vi "IMU Get Yaw Flat.vi"(7 "Alignment Angle":dbl=nan, 8 "error in (no error)":errorcluster, 10 "Units":enum16{"Radians", "Degrees"}(ring)) -> (0 "error out":errorcluster, 2 "timestamp out":i64, 3 "yaw":dbl(graph))   [LabVIEW 2023, in "MrcLib.lvlib"]
doc: "Return the yaw of the built-in sensor in the indicated units assuming it is mounted flat/horizontal relative to the ground (very common). To align with a existing coordinate system, make a call passing in the expected alignment angle."
uses:
  <vilib>/MRC/MrcLib.lvlib
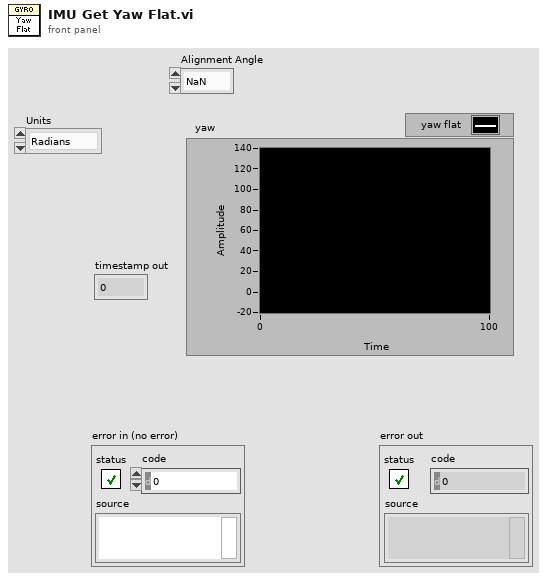
[diagram p1: front panel]
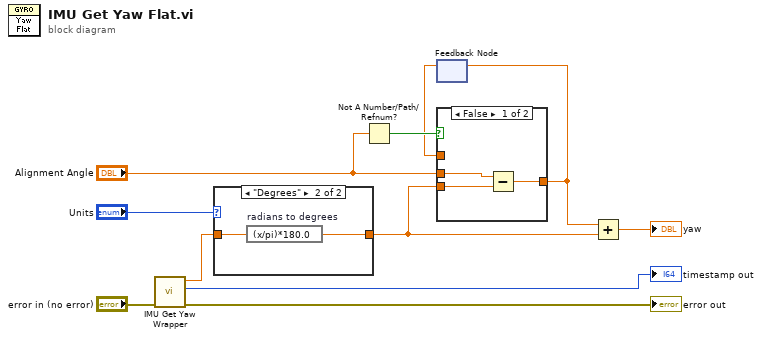
[diagram p0: block diagram]
diagram:
  n1 = call-poly <vilib>:"IMU Get Yaw Wrapper.vi"("error in (no error)"="error in (no error)") -> ("error out"=→"error out":errorcluster, "timestamp out"=→"timestamp out":i64, "yaw out"=w2:dbl)  [unwired: 8 in]
  n2 = case shown="\"Degrees\"" "Units" {
    tunnel: w2 -> [w12 w14]
    tunnel: [w12 w13] -> w1
    frame "Radians", Default {
    }
    frame "Degrees" {
      n3 = expression code="(x/pi)*180.0" "radians to degrees"(w14) -> (w13:dbl)
    }
  }
  n4 = Not A Number/Path/Refnum?(number/path/refnum="Alignment Angle") -> (NaN/Path/Refnum?=w8:bool)
  n5 = feedback #1() -> (w6:dbl)  [unwired: 1 in]
  n6 = case shown="False" w8 {
    tunnel: w1 -> [w17 _]
    tunnel: "Alignment Angle" -> [w16 _]
    tunnel: [w15 w18] -> w5
    tunnel: w6 -> [_ w18]
    frame False {
      n7 = Subtract(x=w16, y=w17) -> (x-y=w15:dbl)
    }
    frame True {
    }
  }
  n8 = feedback-in #1(w5) -> ()
  n9 = Add(x=w5, y=w1) -> (x+y=→"yaw":dbl)
